vi "DAQ Variable Control.vi"(8 "error in (no error)":errorcluster, 9 "Cell String 2":string, 10 "Test Object":T1, 11 "Write to AO":dbl) -> (0 "error out":errorcluster, 1 "Scaled Analog Input":dbl[](array[numeric]), 2 "Rotation/Torque":dbl, 3 "Boolean":bool)   [LabVIEW 2021]
uses:
  TypeDefs/Tester Object.ctl
  <vilib>/NI/Modbus Library/API/Master/Modbus Master.lvclass
  <vilib>/NI/Modbus Library/API/Slave/Modbus Slave.lvclass
  Motor/Motor.lvclass
  Elevator/Elevator.lvclass
  Modbus_Master/Modbus_Master.lvclass
  ServoDrive/ServoDrive.lvclass
  TypeDefs/UIControlReferences.ctl
  TypeDefs/Devices Cluster.ctl
  Modbus/Modbus Cluster.ctl
  Modbus/Modbus Address Cluster.ctl
  DAQNav/DAQNav Cluster.ctl
  DAQNav/Analog Cluster.ctl
  Device Context/Device Context Cluster.ctl
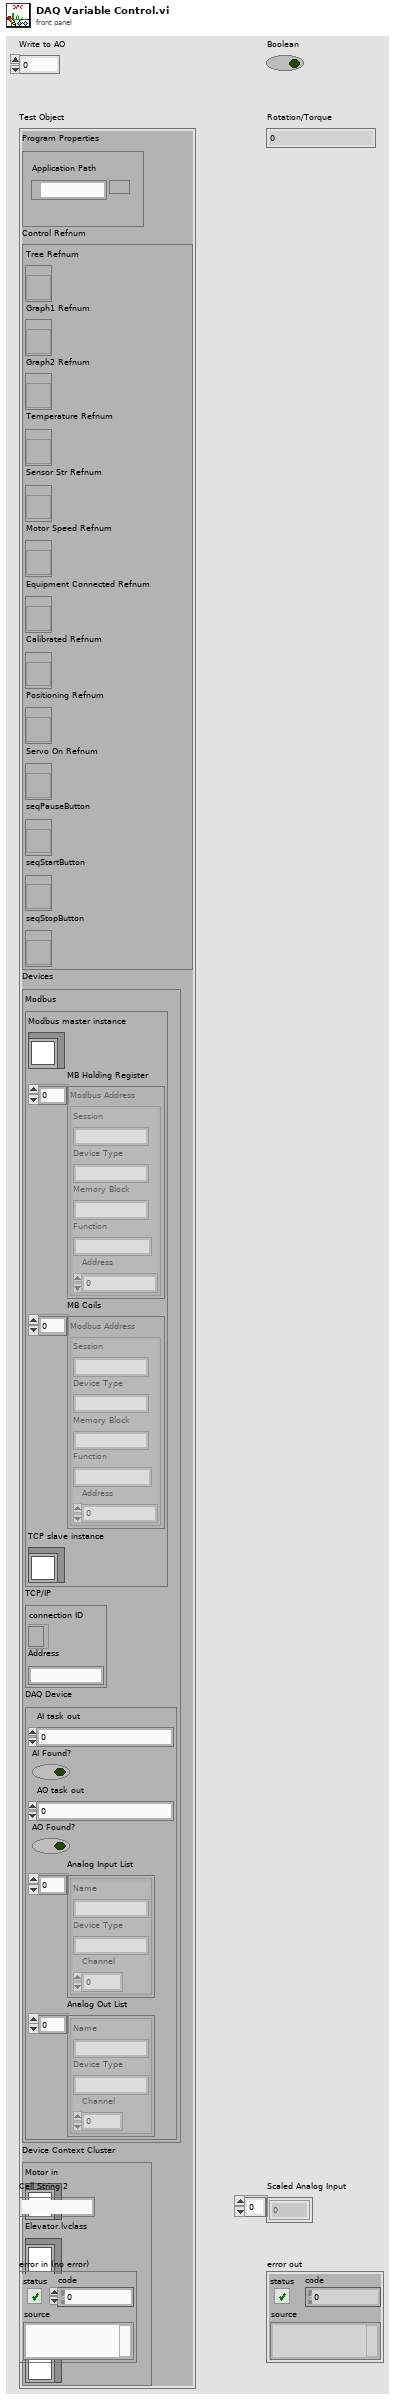
[diagram p1: front panel]
types:
  T1 = typedef "Tester Object.ctl" = cluster{"Program Properties":cluster{"Application Path":path}, "Control Refnum":T2, "Devices":T3, "Device Context Cluster":T8}
  T2 = typedef "UIControlReferences.ctl" = cluster{"Tree Refnum ":refnum<vi>, "Graph1 Refnum":refnum<vi>, "Graph2 Refnum":refnum<vi>, "Temperature Refnum":refnum<vi>, "Sensor Str Refnum":refnum<vi>, "Motor Speed Refnum":refnum<vi>, "Equipment Connected Refnum":refnum<vi>, "Calibrated Refnum":refnum<vi>, "Positioning Refnum":refnum<vi>, "Servo On Refnum":refnum<vi>, "seqPauseButton":refnum<vi>, "seqStartButton":refnum<vi>, "seqStopButton":refnum<vi>}
  T3 = typedef "Devices Cluster.ctl" = cluster{"Modbus":T4, "TCP/IP":cluster{"connection ID":refnum<k5>, "Address":string}, "DAQ Device":T6}
  T4 = typedef "Modbus Cluster.ctl" = cluster{"Modbus master instance":refnum<class "Modbus Master.lvclass">, "MB Holding Register":T5[], "MB Coils":T5[], "TCP slave instance":refnum<class "Modbus Slave.lvclass">}
  T5 = typedef "Modbus Address Cluster.ctl" = cluster{"Session":string, "Device Type":string, "Memory Block":string, "Function":string, "Address":u16}
  T6 = typedef "DAQNav Cluster.ctl" = cluster{"AI task out":i32, "AI Found?":bool, "AO task out":i32, "AO Found?":bool, "Analog Input List":T7[], "Analog Out List":T7[]}
  T7 = typedef "Analog Cluster.ctl" = cluster{"Name":string, "Device Type":string, "Channel":i32}
  T8 = typedef "Device Context Cluster.ctl" = cluster{"Motor in":refnum<class "Motor.lvclass">, "Elevator.lvclass":refnum<class "Elevator.lvclass">, "Modbus_Master.lvclass":refnum<class "Modbus_Master.lvclass">, "ServoDrive.lvclass":refnum<class "ServoDrive.lvclass">}
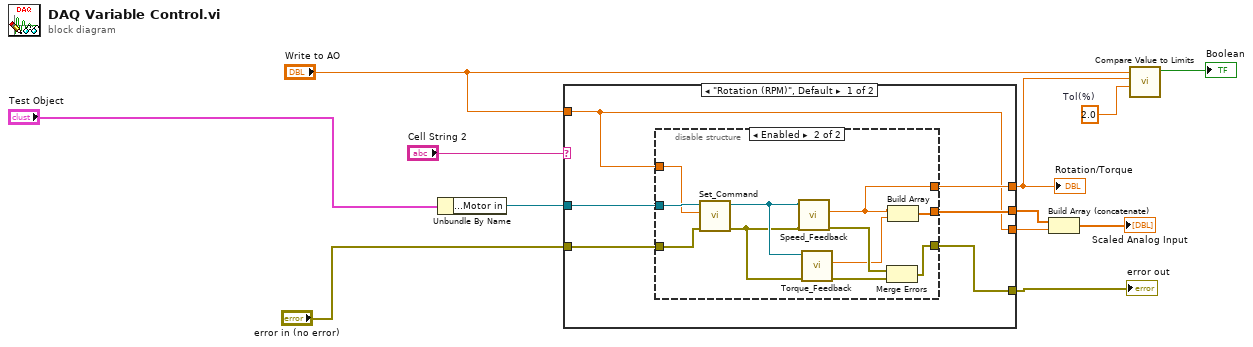
[diagram p0: block diagram]
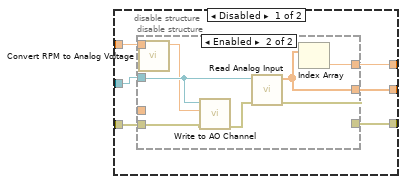
[diagram p2: hidden frame]
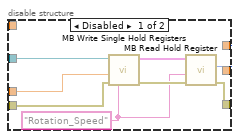
[diagram p3: hidden frame]
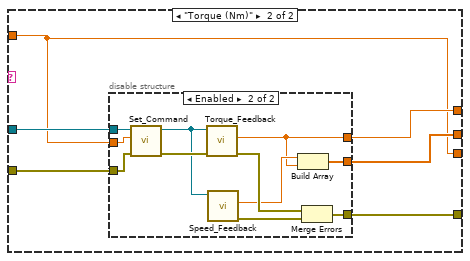
[diagram p4: hidden frame]
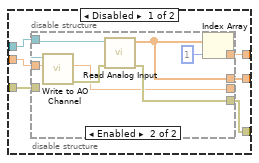
[diagram p5: hidden frame]
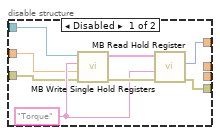
[diagram p6: hidden frame]
diagram:
  w4 = 2.0  # Tol(%)
  n1 = Unbundle By Name("Test Object") -> ("Device Context Cluster.Motor in"=w10:refnum<class "Motor.lvclass">)
  n2 = case shown="\"Rotation (RPM)\", Default" "Cell String 2" {
    tunnel: w10 -> [w15 w57]
    tunnel: "error in (no error)" -> [w16 w54]
    tunnel: [w17 w56] -> w11
    tunnel: [w18 w55] -> w12
    tunnel: "Write to AO" -> [w13 w52]
    tunnel: [w14 w53] -> w2
    tunnel: [w13 w52] -> w3
    frame "Rotation (RPM)", Default {
      n3 = disable-structure shown="Enabled" {
        disable-tunnel: [w24 w45] -> w18
        disable-tunnel: [w23 w42] -> w17
        disable-tunnel: w16 -> [w22 w49]
        disable-tunnel: w15 -> [w21 w51]
        disable-tunnel: [w20 w41] -> w14
        disable-tunnel: w13 -> [w19 w50]
        frame Disabled {
          n4 = disable-structure shown="Enabled" {
            disable-tunnel: w21 -> [w29 w35]
            disable-tunnel: [w28 w40] -> w24
            disable-tunnel: [w27 w39] -> w23
            disable-tunnel: _ -> [w26 _]
            disable-tunnel: w22 -> [w25 w37]
            disable-tunnel: [_ w38] -> w20
            disable-tunnel: w19 -> [_ w34]
            frame Disabled {
              w30 = "Rotation_Speed" ("Control Variable")
              n5 = call "MB Write Single Hold Registers.vi"("error in (no error)"=w25, "Write Hold Register"=w26, "Control Variable"=w30, "Devices"=w29) -> ("error out"=w32:errorcluster, "Devices out"=w31:T4)  [unwired: 6 in]
              n6 = call "MB Read Hold Register.vi"("error in"=w32, "Key"=w30, "Devices"=w31) -> ("error out"=w28:errorcluster, "Register value"=w27:u16)  [unwired: 6 in, 1 out]
            }
            frame Enabled {
              n7 = call "Convert RPM to Analog Voltage.vi"("Write to AO"=w34) -> ("Numeric"=w33:dbl)  [unwired: 10 in]
              n8 = call "Write to AO Channel.vi"("error in"=w37, "ctrlMotorControl"=w33, "DAQ Device"=w35) -> ("error out"=w36:errorcluster)  [unwired: 6 in, 2 out]
              n9 = call "Read Analog Input.vi"("error in (no error)"=w36, "Devices.DAQ Device"=w35) -> ("error out"=w40:errorcluster, "Scaled Analog Input"=w38:dbl[])  [unwired: 7 in, 1 out]
              n10 = Index Array(array=w38) -> (element=w39:dbl)  [unwired: 1 in]
            }
          }
        }
        frame Enabled {
          n11 = call "Set_Command.vi"("error in (no error)"=w49, "Motor Control"=w50, "Motor in"=w51) -> ("error out"=w46:errorcluster, "Motor out"=w47:refnum<class "Motor.lvclass">)  [unwired: 7 in]
          n12 = call "Speed_Feedback.vi"("error in (no error)"=w46, "Motor in"=w47) -> ("error out"=w48:errorcluster, "Actual Speed"=w42:dbl)  [unwired: 7 in, 1 out]
          n13 = call "Torque_Feedback.vi"("error in (no error)"=w46, "Motor in"=w47) -> ("error out"=w44:errorcluster, "Actual Torque"=w43:dbl)  [unwired: 7 in, 1 out]
          n14 = Merge Errors(w48, w44) -> (w45:errorcluster)
          n15 = Build Array(w42, w43) -> (w41:dbl[])
        }
      }
    }
    frame "Torque (Nm)" {
      n16 = disable-structure shown="Enabled" {
        disable-tunnel: w57 -> [w63 w90]
        disable-tunnel: [w62 w81] -> w56
        disable-tunnel: [w61 w84] -> w55
        disable-tunnel: w54 -> [w60 w88]
        disable-tunnel: [w59 w80] -> w53
        disable-tunnel: w52 -> [w58 w89]
        frame Disabled {
          n17 = disable-structure shown="Enabled" {
            disable-tunnel: w63 -> [w68 w73]
            disable-tunnel: [w67 w77] -> w62
            disable-tunnel: [w66 w79] -> w61
            disable-tunnel: w60 -> [w65 _]
            disable-tunnel: w58 -> [w64 w75]
            disable-tunnel: [_ w76] -> w59
            disable-tunnel: [_ w72] -> _
            frame Disabled {
              w69 = "Torque" ("Control Variable")
              n18 = call "MB Write Single Hold Registers.vi"("error in (no error)"=w65, "Write Hold Register"=w64, "Control Variable"=w69, "Devices"=w68) -> ("error out"=w71:errorcluster, "Devices out"=w70:T4)  [unwired: 6 in]
              n19 = call "MB Read Hold Register.vi"("error in"=w71, "Key"=w69, "Devices"=w70) -> ("error out"=w66:errorcluster, "Register value"=w67:u16)  [unwired: 6 in, 1 out]
            }
            frame Enabled {
              n20 = call "Write to AO Channel.vi"("ctrlMotorControl"=w75, "DAQ Device"=w73) -> ("error out"=w74:errorcluster, "ctrlMotorControl written"=w72:dbl)  [unwired: 7 in, 1 out]
              n21 = call "Read Analog Input.vi"("error in (no error)"=w74, "Devices.DAQ Device"=w73) -> ("error out"=w79:errorcluster, "Scaled Analog Input"=w76:dbl[])  [unwired: 7 in, 1 out]
              n22 = Index Array(array=w76, index=1) -> (element=w77:dbl)
            }
          }
        }
        frame Enabled {
          n23 = call "Set_Command.vi"("error in (no error)"=w88, "Motor Control"=w89, "Motor in"=w90) -> ("error out"=w87:errorcluster, "Motor out"=w83:refnum<class "Motor.lvclass">)  [unwired: 7 in]
          n24 = call "Torque_Feedback.vi"("error in (no error)"=w87, "Motor in"=w83) -> ("error out"=w86:errorcluster, "Actual Torque"=w81:dbl)  [unwired: 7 in, 1 out]
          n25 = call "Speed_Feedback.vi"("Motor in"=w83) -> ("error out"=w85:errorcluster, "Actual Speed"=w82:dbl)  [unwired: 8 in, 1 out]
          n26 = Build Array(w82, w81) -> (w80:dbl[])
          n27 = Merge Errors(w86, w85) -> (w84:errorcluster)
        }
      }
    }
  }
  "Rotation/Torque" <- w11
  "error out" <- w12
  n28 = Build Array (concatenate)(w2, w3) -> (→"Scaled Analog Input":dbl[])
  n29 = call "Compare Value to Limits.vi"("Tol(%)"=w4, "Variable Monitored"=w11, "Write to AO"="Write to AO") -> ("Boolean"=→"Boolean":bool)  [unwired: 8 in]
